vi "Alarms.SetAll.vi"(7 "Station.ID":string, 8 "error in (no error)":errorcluster, 10 "Alarms":T1[](array[typedef]) {"Delay" format="%.2f"; "Low Limit" format="%.2f"; "High Limit" format="%.2f"}, 11 "ListBox in":refnum<vi>) -> (0 "error out":errorcluster)   [LabVIEW 2015, in "Single Station Execution.lvlib"]
uses:
  Single Station Execution.lvlib
  Types/Config.AlarmSettings.ctl
  <vilib>/NI Veristand/Execution/Alarm/NI_VS Alarm ExecutionAPI.lvlib
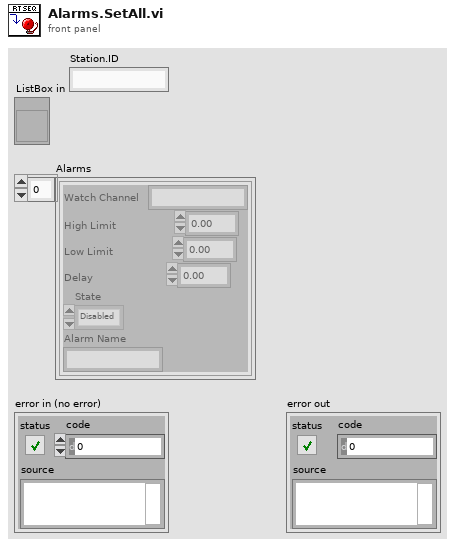
[diagram p1: front panel]
types:
  T1 = typedef "Single Station Execution.lvlib/Config.AlarmSettings.ctl" = cluster{"Watch Channel":string, "High Limit":dbl, "Low Limit":dbl, "Delay":dbl, "State":enum16{"Disabled", "Enabled", "Tripped", "Delayed Trip", "Indicate"}, "Alarm Name":string}
  T2 = enum16{"Disabled", "Enabled", "Tripped", "Delayed Trip", "Indicate"}
  T3 = typedef "NI_VS Alarm ExecutionAPI.lvlib/AlarmAPI.ctl" = refnum<k24>
  T4 = typedef "NI_VS Alarm ExecutionAPI.lvlib/AlarmInfo.ctl" = cluster{"Watch Channel":string, "High Limit Constant":bool, "High Limit Channel":string, "High Limit":dbl, "Low Limit Constant":bool, "Low Limit Channel":string, "Low Limit":dbl, "Procedure Name":string, "Delay":dbl, "Trip Value":dbl, "Priority":enum16{"Low", "Medium", "High"}, "State":enum16{"Disabled", "Enabled", "Tripped", "Delayed Trip", "Indicate"}, "Mode":enum16{"Normal", "Indicate Only"}, "Group Number":u32, "Priority Number":u32, "Name":string, "Full Name":string}
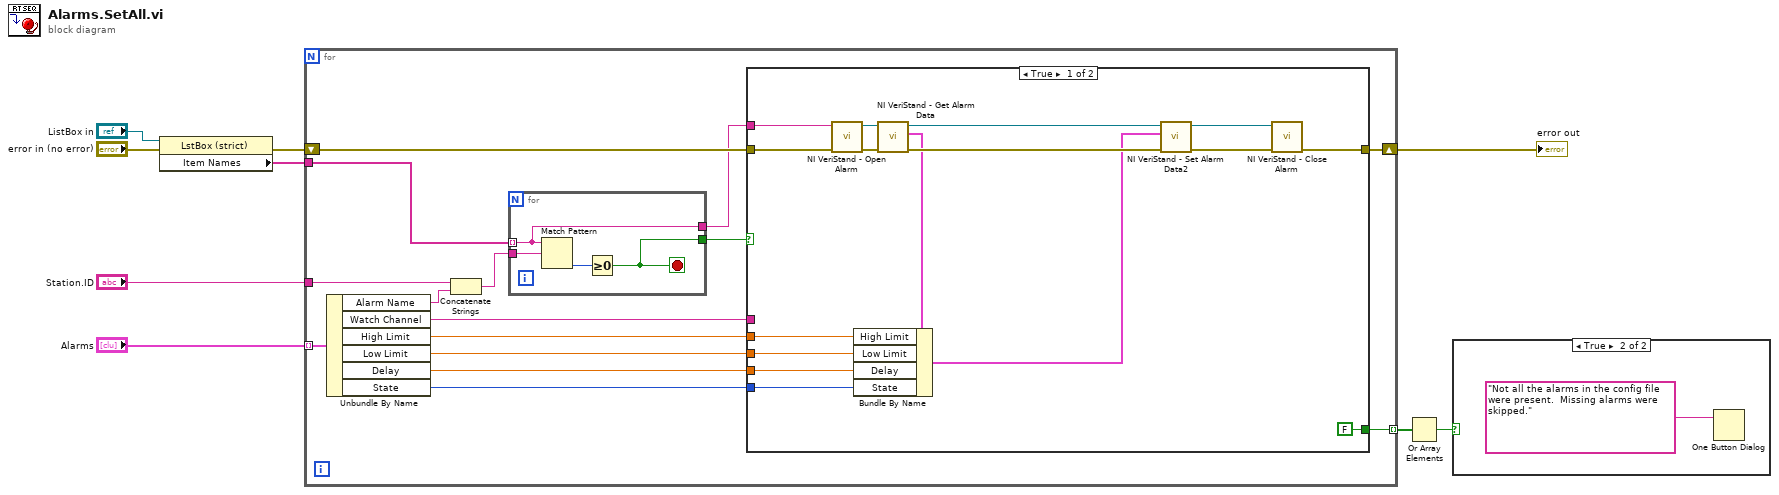
[diagram p0: block diagram]
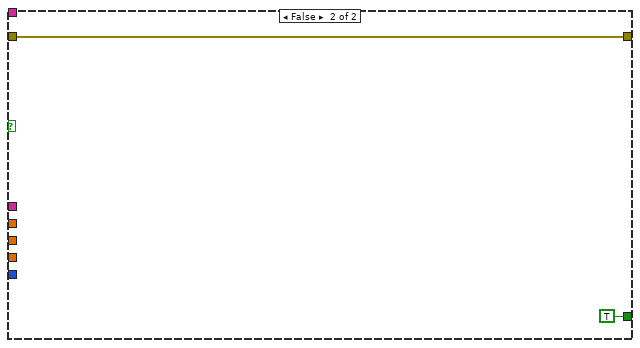
[diagram p3: hidden frame]
diagram:
  n1 = property class="LstBox (strict)"(reference="ListBox in", error in="error in (no error)") -> (error out=w4:errorcluster, "Item Names"=w6:string[])  [unwired: 1 out]
  n2 = for {
    shift-right: [w22] -> w7
    shift-left: w4 -> [w23]
    tunnel: "Alarms" -> [w24] mode=indexing
    tunnel: w6 -> [w14]
    tunnel: [w16] -> w8 mode=indexing
    tunnel: "Station.ID" -> [w15]
    n3 = Unbundle By Name(w24) -> ("Alarm Name"=w11:string, "Watch Channel"=w17:string, "High Limit"=w18:dbl, "Low Limit"=w19:dbl, "Delay"=w20:dbl, "State"=w21:T2)
    n4 = Concatenate Strings(w15, w11) -> (w13:string)
    n5 = for {
      tunnel: w14 -> [w26] mode=indexing
      tunnel: w13 -> [w28]
      tunnel: [w26] -> w10
      tunnel: [w25] -> w12
      stop <- w25 stop-if-true
      n6 = Match Pattern(string=w26, regular expression=w28) -> (offset past match=w27:i32)  [unwired: 1 in, 3 out]
      n7 = Greater Or Equal To 0?(x=w27) -> (x >= 0?=w25:bool)
    }
    n8 = case shown="True" w12 {
      tunnel: w23 -> [w44 w46]
      tunnel: [w40 w46] -> w22
      tunnel: w10 -> [w31 _]
      tunnel: w21 -> [w35 _]
      tunnel: w20 -> [w34 _]
      tunnel: w19 -> [w33 _]
      tunnel: w18 -> [w32 _]
      tunnel: w17 -> [_ _]
      tunnel: [FALSE TRUE] -> w16
      frame True {
        n9 = call <vilib>:"NI VeriStand - Open Alarm.vi"("error in (no error)"=w44, "Alarm Name"=w31) -> ("error out"=w43:errorcluster, "Alarm"=w39:T3)  [unwired: 8 in]
        n10 = call <vilib>:"NI VeriStand - Get Alarm Data.vi"("error in (no error)"=w43, "Alarm in"=w39) -> ("error out"=w42:errorcluster, "Alarm Data"=w36:T4, "Alarm out"=w38:T3)  [unwired: 7 in]
        n11 = Bundle By Name(cluster=w36, "High Limit"=w32, "Low Limit"=w33, "Delay"=w34, "State"=w35) -> (w30:T4)
        n12 = call <vilib>:"NI VeriStand - Set Alarm Data2.vi"("error in (no error)"=w42, "Alarm Data"=w30, "Alarm in"=w38) -> ("error out"=w41:errorcluster, "Alarm out"=w37:T3)  [unwired: 7 in]
        n13 = call <vilib>:"NI VeriStand - Close Alarm.vi"("error in (no error)"=w41, "Alarm"=w37) -> ("error out"=w40:errorcluster)  [unwired: 9 in]
      }
      frame False {
      }
    }
  }
  "error out" <- w7
  n14 = Or Array Elements(Boolean array=w8) -> (logical OR=w9:bool)
  n15 = case shown="True" w9 {
    frame False {
    }
    frame True {
      n16 = One Button Dialog(message="Not all the alarms in the config file were present.  Missing alarms were skipped.") -> ()  [unwired: 1 in, 1 out]
    }
  }
